vi "RDC-Lin-Calc_capacitance.vi"(11 "Open Probe reading":T1={"Frequency"=array[2001 elements], "Reflection'"=array[2001 elements], "Reflection''"=array[2001 elements], "Permativity'"=array[2001 elements], "Permativity''"=array[2001 elements], "Conductivity"=array[2001 elements], "Loss Tangent"=array[2001 elements], "Resistance"=[], "Reactance"=[]}) -> (1 "Cap array":dbl[](array[numeric]), 2 "C0":dbl format="%#_6p")   [LabVIEW 2020, in "RDC-Reflection_Data_Computation.lvlib"]
doc: "Computes the capacitance per frequency from an open-probe Common Format cluster and returns it as Cap array, with its average as C0."
uses:
  RDC-Reflection_Data_Computation.lvlib
  Reflector/RFH-common_data_format.ctl
  9ba1e4c3-b37a-4ae0-8c78-9d1f2c3753c0.vi
  Reflector/RFH-Reflection_File_Handler.lvlib
panel:
  out "Waveform Graph":dbl[](graph)
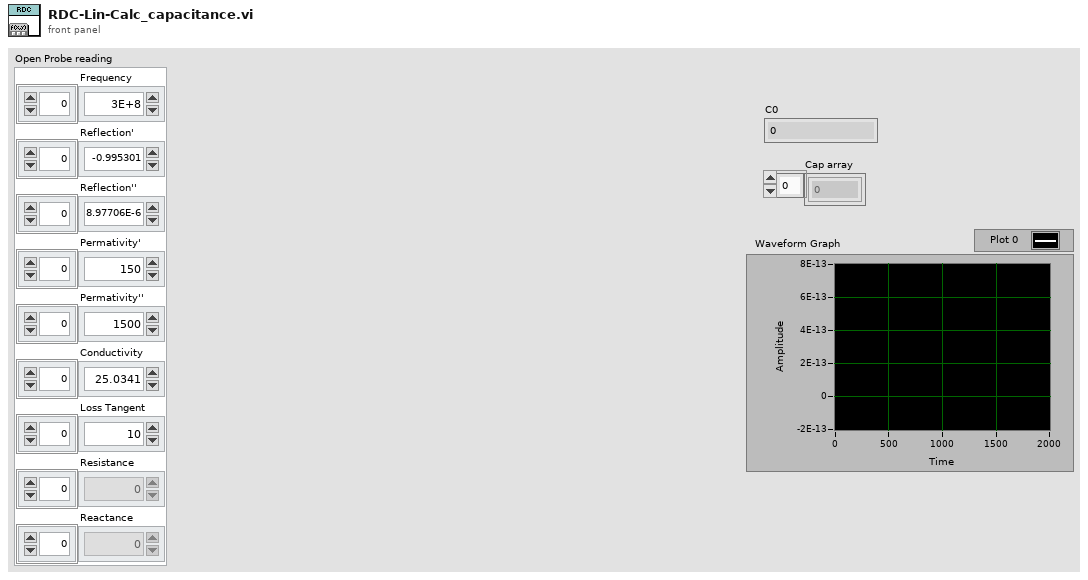
[diagram p1: front panel]
types:
  T1 = typedef "RFH-Reflection_File_Handler.lvlib/RFH-common_data_format.ctl" = cluster{"Frequency":dbl[], "Reflection'":dbl[], "Reflection''":dbl[], "Permativity'":dbl[], "Permativity''":dbl[], "Conductivity":dbl[], "Loss Tangent":dbl[], "Resistance":dbl[], "Reactance":dbl[]}
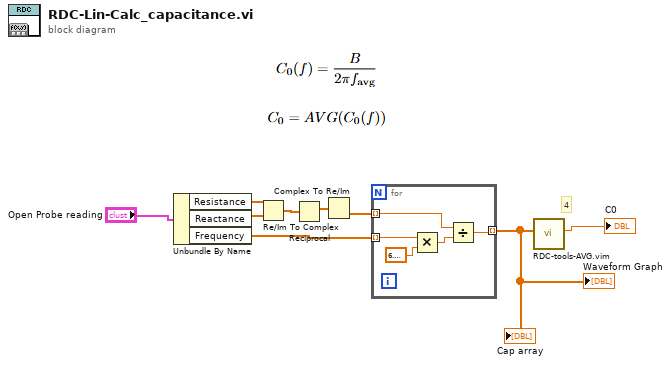
[diagram p0: block diagram]
diagram:
  # "4"
  n1 = Unbundle By Name("Open Probe reading") -> ("Resistance"=w6:dbl[], "Reactance"=w5:dbl[], "Frequency"=w9:dbl[])
  n2 = Re/Im To Complex(1:w5, 2:w6) -> (0:w4:cdb[])
  n3 = Reciprocal(x=w4) -> (1/x=w3:cdb[])
  n4 = Complex To Re/Im(x + iy=w3) -> (y=w8:dbl[])  [unwired: 1 out]
  n5 = for {
    tunnel: w8 -> [w10] mode=indexing
    tunnel: w9 -> [w13] mode=indexing
    tunnel: [w11] -> w1 mode=indexing
    n6 = Multiply(x=w13, y=6.283185307179586) -> (x*y=w14:dbl)
    n7 = Divide(x=w10, y=w14) -> (x/y=w11:dbl)
  }
  "Cap array" <- w1
  "Waveform Graph" <- w1
  n8 = call "RDC-tools-AVG.vim"("Data Array"=w1) -> ("AVG"=→"C0":dbl)  [unwired: 10 in]
